vi "Check Parameter.vi"(6 "Options in":T1={"DbType"=-1, "Direction"=-1, "Size"=-1, "Precision"=255, "Scale"=255} {"Direction" items=["Input"=1, "Output"=2, "InputOutput"=3, "ReturnValue"=6]; "DbType" items=["AnsiString"=0, "Binary"=1, "Byte"=2, "Boolean"=3, "Currency"=4, "Date"=5, "DateTime"=6, "Decimal"=7, "Double"=8, "Guid"=9, "Int16"=10, "Int32"=11, "Int64"=12, "Object"=13, "SByte"=14, "Single"=15, "String"=16, "Time"=17, "UInt16"=18, "UInt32"=19, "UInt64"=20, "VarNumeric"=21, "AnsiStringFixedLength"=22, "StringFixedLength"=23, "Xml"=25, "DateTime2"=26, "DateTimeOffset"=27]}, 8 "error in (no error)":errorcluster, 9 "value in":variant, 10 "name in":string, 11 "PostgresqlConnection in":refnum<class "DBC.lvclass">) -> (0 "error out":errorcluster, 1 "value out":variant, 2 "name out":string, 3 "PostgresqlConnection out":refnum<class "DBC.lvclass">, 4 "Options out":T1={"DbType"=-1, "Direction"=-1, "Size"=-1, "Precision"=255, "Scale"=255} {"Direction" items=["Input"=1, "Output"=2, "InputOutput"=3, "ReturnValue"=6]; "DbType" items=["AnsiString"=0, "Binary"=1, "Byte"=2, "Boolean"=3, "Currency"=4, "Date"=5, "DateTime"=6, "Decimal"=7, "Double"=8, "Guid"=9, "Int16"=10, "Int32"=11, "Int64"=12, "Object"=13, "SByte"=14, "Single"=15, "String"=16, "Time"=17, "UInt16"=18, "UInt32"=19, "UInt64"=20, "VarNumeric"=21, "AnsiStringFixedLength"=22, "StringFixedLength"=23, "Xml"=25, "DateTime2"=26, "DateTimeOffset"=27]})   [LabVIEW 2020, in "ORM_sqlite_jdp.lvlib" / "DBC.lvclass"]
uses:
  DBC.lvclass
  <vilib>/Viviota/shared/ORM.lvlibp/DbConnection/DbConnection.lvclass
  <vilib>/regexp/Match Regular Expression.xnode
  DBC.lvclass/DBC.ctl
  <vilib>/JDP Science/JSONtext/JSONtext.lvlib
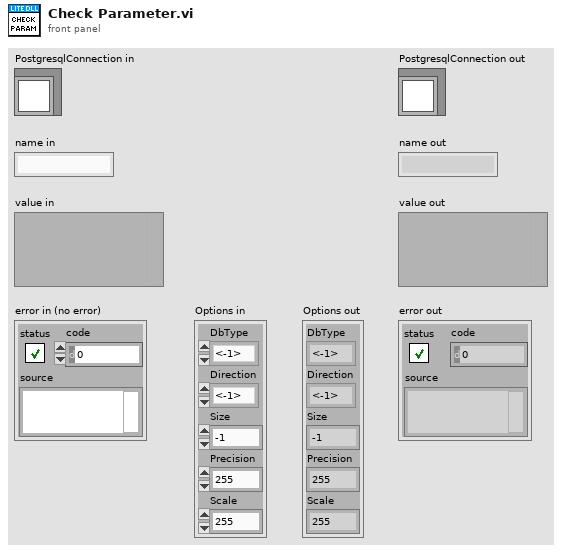
[diagram p1: front panel]
types:
  T1 = cluster{"DbType":i32, "Direction":i32, "Size":i32, "Precision":u8, "Scale":u8}
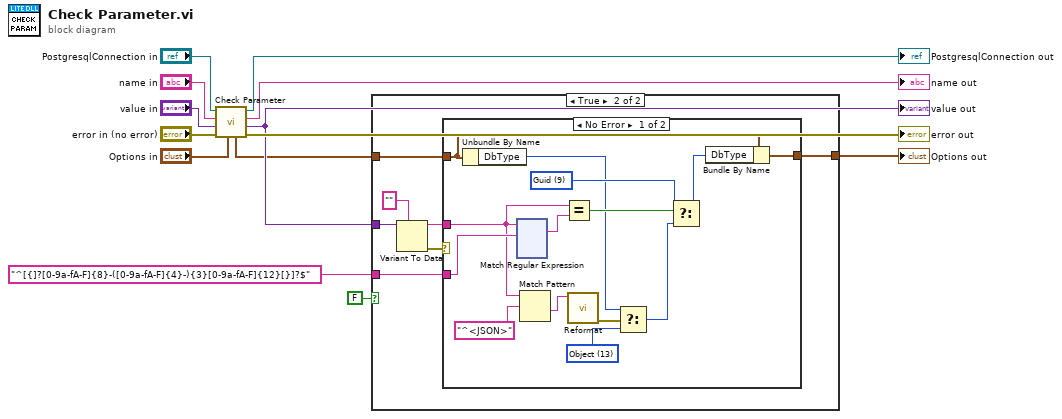
[diagram p0: block diagram]
diagram:
  n1 = call-parent "Check Parameter.vi"("Options in"="Options in", "error in (no error)"="error in (no error)", "value in"="value in", "name in"="name in", "DbConnection in"="PostgresqlConnection in") -> ("error out"=→"error out":errorcluster, "value out"=w6:variant, "name out"=→"name out":string, "DbConnection out"=→"PostgresqlConnection out":refnum<class "DBC.lvclass">, "Options out"=w4:T1)  [unwired: 2 in]
  "value out" <- w6
  n2 = case shown="True" FALSE {
    tunnel: w6 -> [_ w21]
    tunnel: "^[{]?[0-9a-fA-F]{8}-([0-9a-fA-F]{4}-){3}[0-9a-fA-F]{12}[}]?$" -> [_ w17]
    tunnel: w4 -> [w14 w16]
    tunnel: [w14 w15] -> w3
    frame False {
      # "Right now we're autoparsing parameters on the pgsql side\nso ignoring this for now (for testing)"
    }
    frame True {
      n3 = Variant To Data(type="", Variant=w21) -> (data=w18:string, error out=w19:errorcluster)  [unwired: 1 in]
      n4 = case shown="No Error" w19 {
        tunnel: w18 -> [w22 _]
        tunnel: w17 -> [w25 _]
        tunnel: w16 -> [w31 w150]
        tunnel: [w30 w150] -> w15
        frame No Error {
          w28 = 13 items=["AnsiString"=0, "Binary"=1, "Byte"=2, "Boolean"=3, "Currency"=4, "Date"=5, "DateTime"=6, "Decimal"=7, "Double"=8, "Guid"=9, "Int16"=10, "Int32"=11, "Int64"=12, "Object"=13, "SByte"=14, "Single"=15, "String"=16, "Time"=17, "UInt16"=18, "UInt32"=19, "UInt64"=20, "VarNumeric"=21, "AnsiStringFixedLength"=22, "StringFixedLength"=23, "Xml"=25, "DateTime2"=26, "DateTimeOffset"=27] ("DbType")
          w33 = 9 items=["AnsiString"=0, "Binary"=1, "Byte"=2, "Boolean"=3, "Currency"=4, "Date"=5, "DateTime"=6, "Decimal"=7, "Double"=8, "Guid"=9, "Int16"=10, "Int32"=11, "Int64"=12, "Object"=13, "SByte"=14, "Single"=15, "String"=16, "Time"=17, "UInt16"=18, "UInt32"=19, "UInt64"=20, "VarNumeric"=21, "AnsiStringFixedLength"=22, "StringFixedLength"=23, "Xml"=25, "DateTime2"=26, "DateTimeOffset"=27] ("DbType")
          n5 = Unbundle By Name(w31) -> ("DbType"=w24:i32)
          n6 = xnode "Match Regular Expression"("input string"=w22, "regular expression"=w25) -> ("whole match"=w35:string)  [unwired: 4 in, 4 out]
          n7 = Match Pattern(string=w22, regular expression="^<JSON>") -> (after substring=w26:string)  [unwired: 1 in, 3 out]
          n8 = Equal?(x=w22, y=w35) -> (x = y?=w34:bool)
          n9 = call <vilib>:"Reformat.vi"("JSON"=w26) -> ("error out"=w29:errorcluster)  [unwired: 7 in, 3 out]
          n10 = Select(t=w24, s=w29, f=w28) -> (s? t:f=w23:i32)
          n11 = Select(t=w33, s=w34, f=w23) -> (s? t:f=w32:i32)
          n12 = Bundle By Name(cluster=w31, "DbType"=w32) -> (w30:T1)
        }
        frame Error {
        }
      }
    }
  }
  "Options out" <- w3
